vi "ZM-launcher.vi"(11 "output_folder":path) -> (0 "error out":errorcluster)   [LabVIEW 2020]
doc: "Interactive launcher of the actor tree. Writes the root's pre-launch settings (output folder for the JSONL files, simulated hardware) and launches the root, then returns; the tree runs until Stop is pressed on the root's panel. An empty output_folder means the output folder next to src. error out is the error of the launch."
uses:
  actors/ZM-ROOT-root/ZM-ROOT-root/ZM-ROOT-root.lvclass
  <vilib>/ActorFramework/Actor/Actor.lvclass
  actors/ZM-ROOT-root/ZM-ROOT-root/ZM-ROOT-PRELAUNCH_SETTINGS.ctl
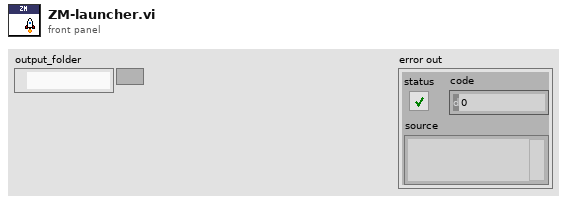
[diagram p1: front panel]
types:
  T1 = typedef "ZM-ROOT-root.lvlib/ZM-ROOT-root.lvclass/ZM-ROOT-PRELAUNCH_SETTINGS.ctl" = cluster{"outputFolder":path, "usePlaceholderHardware":bool}
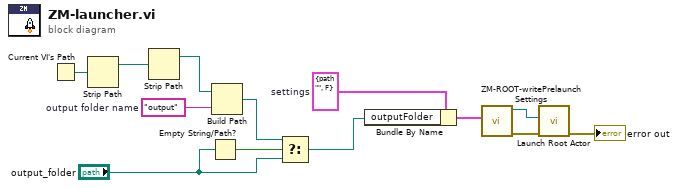
[diagram p0: block diagram]
diagram:
  w10 = "output"  # output folder name
  w5 = T1 {"outputFolder"=path "", "usePlaceholderHardware"=FALSE}  # settings
  n1 = Current VI's Path() -> (path=w13:path)
  n2 = Strip Path(path=w13) -> (stripped path=w12:path)  [unwired: 1 out]
  n3 = Strip Path(path=w12) -> (stripped path=w11:path)  [unwired: 1 out]
  n4 = Empty String/Path?(string/path="output_folder") -> (empty?=w8:bool)
  n5 = Build Path(base path=w11, name or relative path=w10) -> (appended path=w9:path)
  n6 = Select(t=w9, s=w8, f="output_folder") -> (s? t:f=w6:path)
  n7 = Bundle By Name(cluster=w5, "outputFolder"=w6) -> (w4:T1)
  n8 = call "ZM-ROOT-writePrelaunchSettings.vi"("settings"=w4) -> ("error out"=w2:errorcluster, "ZM-ROOT-root out"=w3:refnum<class "ZM-ROOT-root.lvclass">)  [unwired: 9 in]
  n9 = call <vilib>:"Launch Root Actor.vi"("error in (no error)"=w2, "Actor"=w3) -> ("error out"=→"error out":errorcluster)  [unwired: 8 in, 1 out]
